vi "conveyor to box.vi"(2 "error in (no error)":errorcluster, 3 "櫃子":i32) -> (0 "error out":errorcluster)   [LabVIEW 2019]
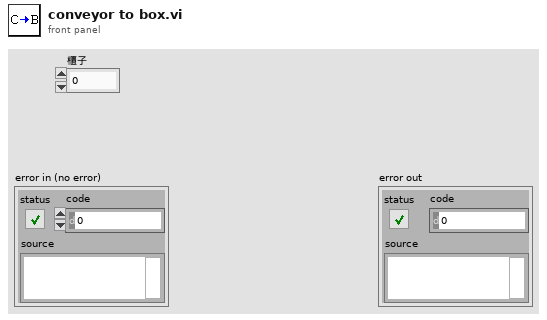
[diagram p1: front panel]
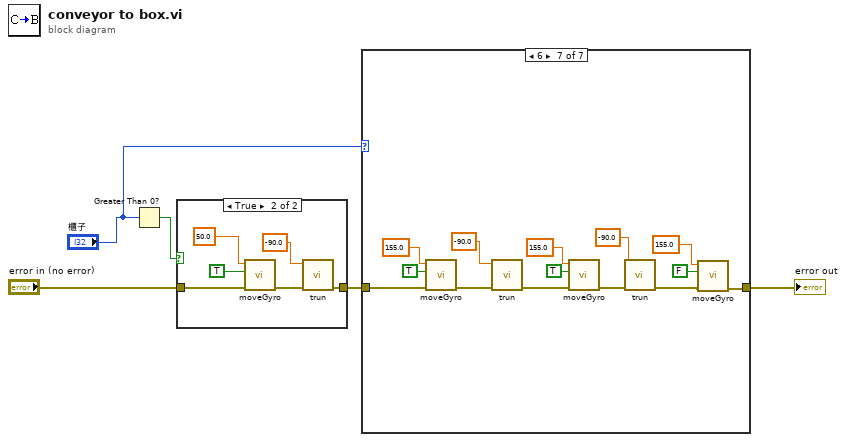
[diagram p0: block diagram]
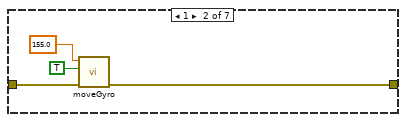
[diagram p4: hidden frame]
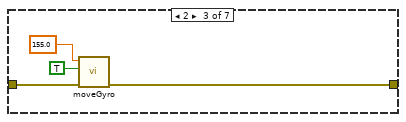
[diagram p5: hidden frame]
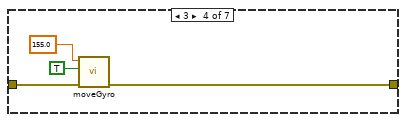
[diagram p6: hidden frame]
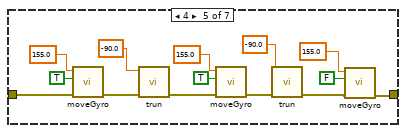
[diagram p7: hidden frame]
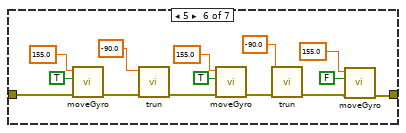
[diagram p8: hidden frame]
diagram:
  n1 = Greater Than 0?(x="櫃子") -> (x > 0?=w4:bool)
  n2 = case shown="True" w4 {
    tunnel: "error in (no error)" -> [w6 w10]
    tunnel: [w6 w11] -> w5
    frame False {
    }
    frame True {
      n3 = call "moveGyro.vi"("error in (no error)"=w10, "タは"=TRUE, "移動距離"=50.0) -> ("error out"=w9:errorcluster)  [unwired: 8 in]
      n4 = call "trun.vi"("error in (no error)"=w9, "旋轉"=-90.0) -> ("error out"=w11:errorcluster)  [unwired: 9 in]
    }
  }
  n5 = case shown="6" "櫃子" {
    tunnel: w5 -> [w13 w16 w20 w24 w36 w50 w64]
    tunnel: [w13 w15 w19 w23 w29 w43 w57] -> w1
    frame 0, Default {
    }
    frame 1 {
      n6 = call "moveGyro.vi"("error in (no error)"=w16, "タは"=TRUE, "移動距離"=155.0) -> ("error out"=w15:errorcluster)  [unwired: 8 in]
    }
    frame 2 {
      n7 = call "moveGyro.vi"("error in (no error)"=w20, "タは"=TRUE, "移動距離"=155.0) -> ("error out"=w19:errorcluster)  [unwired: 8 in]
    }
    frame 3 {
      n8 = call "moveGyro.vi"("error in (no error)"=w24, "タは"=TRUE, "移動距離"=155.0) -> ("error out"=w23:errorcluster)  [unwired: 8 in]
    }
    frame 4 {
      n9 = call "moveGyro.vi"("error in (no error)"=w36, "タは"=TRUE, "移動距離"=155.0) -> ("error out"=w35:errorcluster)  [unwired: 8 in]
      n10 = call "trun.vi"("error in (no error)"=w35, "旋轉"=-90.0) -> ("error out"=w31:errorcluster)  [unwired: 9 in]
      n11 = call "moveGyro.vi"("error in (no error)"=w31, "タは"=TRUE, "移動距離"=155.0) -> ("error out"=w32:errorcluster)  [unwired: 8 in]
      n12 = call "trun.vi"("error in (no error)"=w32, "旋轉"=-90.0) -> ("error out"=w28:errorcluster)  [unwired: 9 in]
      n13 = call "moveGyro.vi"("error in (no error)"=w28, "タは"=FALSE, "移動距離"=155.0) -> ("error out"=w29:errorcluster)  [unwired: 8 in]
    }
    frame 5 {
      n14 = call "moveGyro.vi"("error in (no error)"=w50, "タは"=TRUE, "移動距離"=155.0) -> ("error out"=w49:errorcluster)  [unwired: 8 in]
      n15 = call "trun.vi"("error in (no error)"=w49, "旋轉"=-90.0) -> ("error out"=w45:errorcluster)  [unwired: 9 in]
      n16 = call "moveGyro.vi"("error in (no error)"=w45, "タは"=TRUE, "移動距離"=155.0) -> ("error out"=w46:errorcluster)  [unwired: 8 in]
      n17 = call "trun.vi"("error in (no error)"=w46, "旋轉"=-90.0) -> ("error out"=w42:errorcluster)  [unwired: 9 in]
      n18 = call "moveGyro.vi"("error in (no error)"=w42, "タは"=FALSE, "移動距離"=155.0) -> ("error out"=w43:errorcluster)  [unwired: 8 in]
    }
    frame 6 {
      n19 = call "moveGyro.vi"("error in (no error)"=w64, "タは"=TRUE, "移動距離"=155.0) -> ("error out"=w63:errorcluster)  [unwired: 8 in]
      n20 = call "trun.vi"("error in (no error)"=w63, "旋轉"=-90.0) -> ("error out"=w59:errorcluster)  [unwired: 9 in]
      n21 = call "moveGyro.vi"("error in (no error)"=w59, "タは"=TRUE, "移動距離"=155.0) -> ("error out"=w60:errorcluster)  [unwired: 8 in]
      n22 = call "trun.vi"("error in (no error)"=w60, "旋轉"=-90.0) -> ("error out"=w56:errorcluster)  [unwired: 9 in]
      n23 = call "moveGyro.vi"("error in (no error)"=w56, "タは"=FALSE, "移動距離"=155.0) -> ("error out"=w57:errorcluster)  [unwired: 8 in]
    }
  }
  "error out" <- w1
